vi "VeristandStart.vi"(1 "error in (no error)":errorcluster, 2 "Open VeriStand Timeout (s)":i32=120) -> (0 "error out":errorcluster)   [LabVIEW 2015, in "ni-veristand-steps-runtime-lib.lvlib"]
uses:
  ni-veristand-steps-runtime-lib.lvlib
  <vilib>/Utility/error.llb/Error Cluster From Error Code.vi
  <vilib>/ErrorRing/Error Ring.xnode
  <vilib>/NI Veristand/Execution/Workspace/NI_VS Workspace ExecutionAPI.lvlib
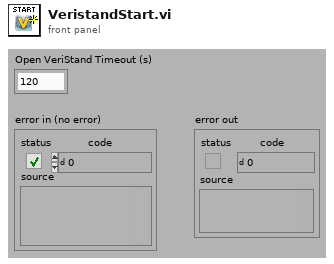
[diagram p1: front panel]
types:
  T1 = typedef "NI_VS Workspace ExecutionAPI.lvlib/WorkspaceAPI.ctl" = refnum<k24>
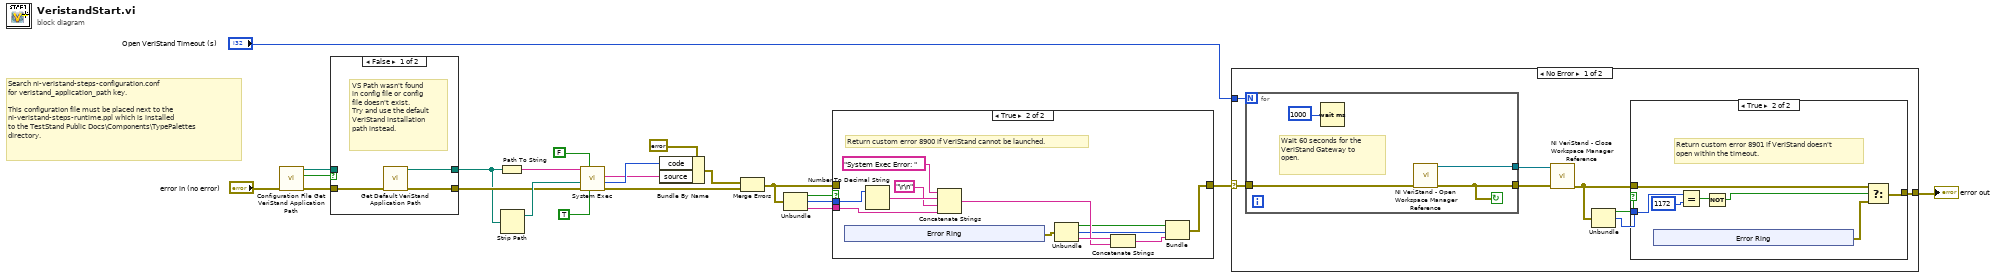
[diagram p0: block diagram]
diagram:
  # "Search ni-veristand-steps-configuration.conf \nfor veristand_application_path key.\n\nThis configuration file must be placed next to the\nni-veristand-steps-runtime.ppl which is installed\nto the TestStand Public Docs\\Components\\TypePalettes\ndirectory."
  n1 = call "Configuration File Get VeriStand Application Path.vi"("error in (no error)"="error in (no error)") -> ("error out"=w12:errorcluster, "Found?"=w10:bool, "VeriStand Application Path"=w11:path)  [unwired: 8 in]
  n2 = case shown="False" w10 {
    tunnel: w12 -> [w25 w26]
    tunnel: w11 -> [_ w27]
    tunnel: [w23 w27] -> w7
    tunnel: [w24 w26] -> w8
    frame False {
      # "VS Path wasn't found\nin config file or config\nfile doesn't exist.\nTry and use the default\nVeriStand installation\npath instead."
      n3 = call "Get Default VeriStand Application Path.vi"("error in (no error)"=w25) -> ("error out"=w24:errorcluster, "Default VeriStand App Path"=w23:path)  [unwired: 9 in]
    }
    frame True {
    }
  }
  n4 = Path To String(path=w7) -> (string=w6:string)
  n5 = Strip Path(path=w7) -> (stripped path=w9:path)  [unwired: 1 out]
  n6 = call <vilib>:"System Exec.vi"("run minimized? (F)"=TRUE, "wait until completion? (T)"=FALSE, "error in (no error)"=w8, "working directory"=w9, "command line"=w6) -> ("error out"=w17:errorcluster, "return code"=w19:i32, "standard error"=w14:string)  [unwired: 3 in, 1 out]
  n7 = Bundle By Name(cluster=errorcluster {"status"=FALSE, "code"=0, "source"=""} ("error in (no error)"), "code"=w19, "source"=w14) -> (w18:errorcluster)
  n8 = Merge Errors(w18, w17) -> (w2:errorcluster)
  n9 = Unbundle(w2) -> ("status"=w5:bool, "code"=w4:i32, "source"=w3:string)
  n10 = case shown="True" w5 {
    tunnel: [w28 w29] -> w1
    tunnel: w4 -> [_ w39]
    tunnel: w3 -> [_ w35]
    tunnel: w2 -> [w28 _]
    frame False {
    }
    frame True {
      # "Return custom error 8900 if VeriStand cannot be launched."
      n11 = xnode "Error Ring"() -> ("error out"=w40:errorcluster)
      n12 = Number To Decimal String(number=w39) -> (decimal integer string=w37:string)  [unwired: 1 in]
      n13 = Concatenate Strings("System Exec Error: " ("string"), w37, "\r\n", w35) -> (w33:string)
      n14 = Unbundle(w40) -> ("status"=w32:bool, "code"=w31:i32, "source"=w34:string)
      n15 = Concatenate Strings(w34, w33) -> (w30:string)
      n16 = Bundle("status"=w32, "code"=w31, w30) -> (w29:cluster{"status":bool, "code":i32, string})  [unwired: 1 in]
    }
  }
  n17 = case shown="No Error" w1 {
    selector: w1 -> [w46 w71]
    tunnel: [w48 w71] -> w16
    tunnel: "Open VeriStand Timeout (s)" -> [w47 _]
    frame No Error {
      n18 = for {
        N: w47 -> [_]
        tunnel: [w68] -> w52
        tunnel: [w69] -> w53
        tunnel: w46 -> [w67]
        stop <- w69 continue-if-true
        # "Wait 60 seconds for the VeriStand Gateway to open."
        n19 = Wait (ms)(milliseconds to wait=u32 1000) -> ()  [unwired: 1 out]
        n20 = call <vilib>:"NI VeriStand - Open Workspace Manager Reference.vi"("error in (no error)"=w67) -> ("error out"=w69:errorcluster, "WorkspaceManager"=w68:T1)  [unwired: 9 in]
      }
      n21 = call <vilib>:"NI VeriStand - Close Workspace Manager Reference.vi"("error in (no error)"=w53, "WorkspaceManager"=w52) -> ("error out"=w50:errorcluster)  [unwired: 9 in]
      n22 = Unbundle(w50) -> ("status"=w51:bool, "code"=w49:i32)  [unwired: 1 out]
      n23 = case shown="True" w51 {
        tunnel: w49 -> [_ w61]
        tunnel: w50 -> [w54 w58]
        tunnel: [w54 w59] -> w48
        frame False {
        }
        frame True {
          # "Return custom error 8901 if VeriStand doesn't\nopen within the timeout."
          n24 = xnode "Error Ring"() -> ("error out"=w55:errorcluster)
          n25 = Equal?(x=w61, y=1172) -> (x = y?=w57:bool)
          n26 = Not(x=w57) -> (.not. x?=w56:bool)
          n27 = Select(t=w58, s=w56, f=w55) -> (s? t:f=w59:errorcluster)
        }
      }
    }
    frame Error {
    }
  }
  "error out" <- w16
